vi "Ramp_Generator.vi"(7 "Delta Time dt (s)":dbl=0.1, 8 "error in (no error)":errorcluster={"status"=FALSE, "code"=0, "source"="\"\""}, 9 "Ramp Rate (units/s)":dbl=10.0, 10 "Target Setpoint":dbl=100.0, 11 "Current Value":dbl) -> (0 "error out":errorcluster, 2 "Target Reached?":bool, 3 "Next Setpoint":dbl)   [LabVIEW 2026]
doc: "Calculates the next setpoint along a controlled ramp, modeled after NI Ramp Gen and Trap Test design patterns."
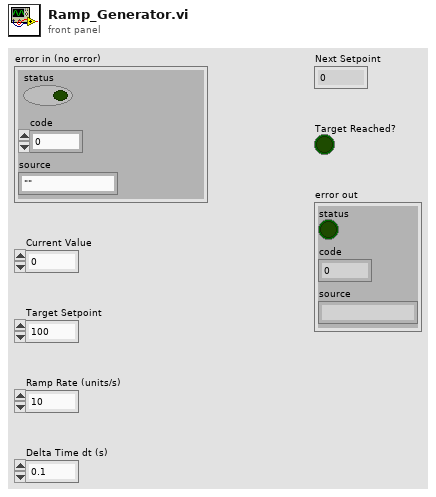
[diagram p1: front panel]
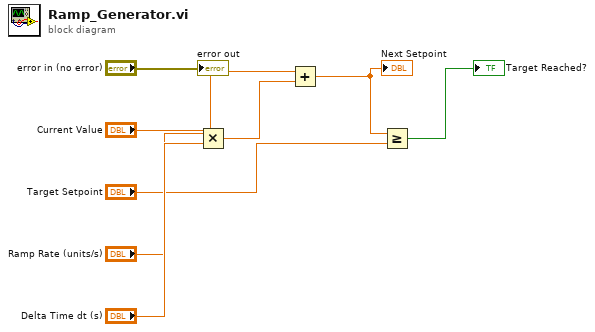
[diagram p0: block diagram]
diagram:
  n1 = Multiply(x="Ramp Rate (units/s)", y="Delta Time dt (s)") -> (x*y=w6:dbl)
  n2 = Add(x="Current Value", y=w6) -> (x+y=w7:dbl)
  "Next Setpoint" <- w7
  n3 = Greater Or Equal?(x=w7, y="Target Setpoint") -> (x >= y?=→"Target Reached?":bool)
  "error out" <- "error in (no error)"
